vi "Module Name--constant.vi"(11 "Module ID":i32=-1) -> (3 "Module Name":string)   [LabVIEW 2020, in "Data Viewer.lvlib"]
doc: "Return the name of the module that owns this VI.\n_____\nBased on DQMH Project Template 7.0.1.1316."
uses:
  Data Viewer.lvlib
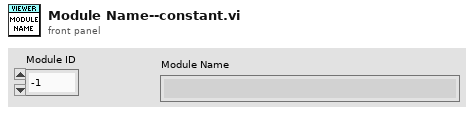
[diagram p1: front panel]
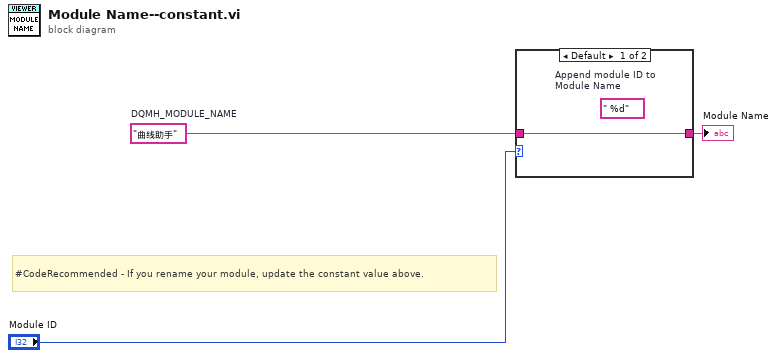
[diagram p0: block diagram]
diagram:
  w1 = "曲线助手"  # DQMH_MODULE_NAME
  # "#CodeRecommended - If you rename your module, update the constant value above."
  n1 = case shown="Default" "Module ID" {
    tunnel: w1 -> [w4 w5]
    tunnel: [w4 w5] -> w3
    frame Default {
      (unwired) " %d"  # Append module ID to  Module Name
    }
    frame ..-1 {
    }
  }
  "Module Name" <- w3
